vi "tdms test.vi"() -> (0 "error out":errorcluster, 3 "Pass":bool)   [LabVIEW 2015, in "tdms logger tests.lvlib"]
uses:
  tdms logger tests.lvlib
  execution/TDMS datalogger runtime.lvclass
  <vilib>/Platform/TimedLoop/XDataNode/timing_clust.ctl
  <vilib>/Platform/TimedLoop/XDataNode/nitl_modes.ctl
  <vilib>/Platform/TimedLoop/XDataNode/wakeup.ctl
  configuration/TDMS datalogger configuration.lvclass/TDMS datalogger configuration.ctl
  <vilib>/NI/Tag Bus/table/data polymorphs/write one/write Boolean.vi
  configuration/Read log directory.vi
  <vilib>/platform/TimedLoop/XDataNode/XDataNode.xnode
  configuration/TDMS datalogger configuration.lvclass
  <vilib>/NI/Tag Bus/table/data table.lvlib
  <vilib>/Platform/TimedLoop/XDataNode/XDNodeRunTimeDep.lvlib
panel:
  out "Property Names Equal?":bool
  out "Property Values Equal?":bool
  out "property values":string[][](array[string])
  out "property names":string[][](array[string])
  out "Data Equal?":bool
  out "Parsed Data":dbl[][](array[numeric])
  out "Channels Equal?":bool
  out "Groups Equal?":bool
  out "channel names":string[](array[string])
  out "group names":string[](array[string])
  out "Data Written":dbl[][](array[numeric])
  in  "iterations":i32=500
  out "max":dbl
  out "min":dbl
  in  "enable state":bool=TRUE
  out "enable found?":bool
  in  "stop":bool
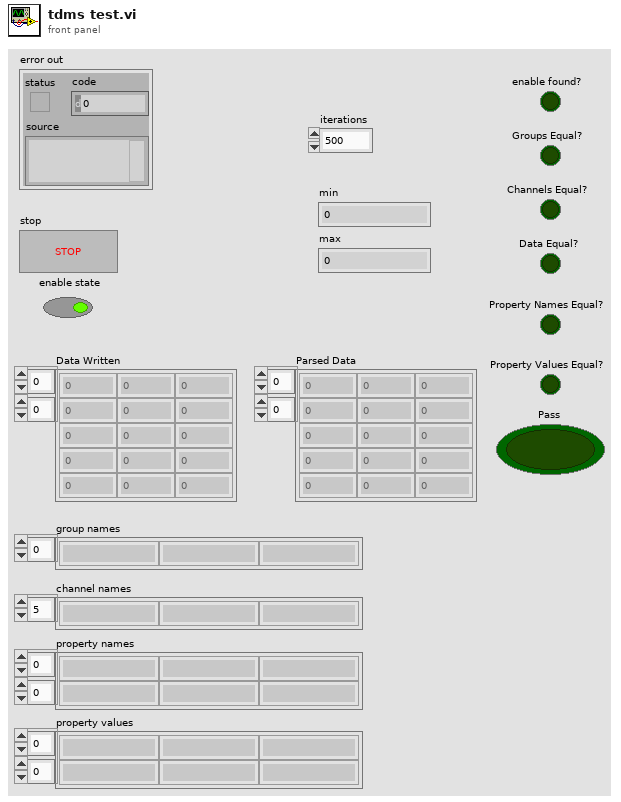
[diagram p1: front panel]
types:
  T1 = typedef "tag bus.lvlib/tag descriptor.lvclass/Data Type.ctl" = enum16{"Double", "Single", "I64", "I32", "I16", "I8", "U64", "U32", "U16", "U8", "Boolean", "String", "Array of Double", "Array of Single", "Array of I64", "Array of I32", "Array of I16", "Array of I8", "Array of U64", "Array of U32", "Array of U16", "Array of U8", "Array of Boolean", "Array of String"}
  T2 = typedef "TBM channel.lvclass/data tables.ctl" = cluster{"input data":T3, "processing parameter":T3, "processing result":T3, "output data":T3}
  T3 = typedef "tag bus.lvlib/dictionary table pair.ctl" = cluster{"data dictionary":refnum<class "data dictionary.lvclass">, "data table":T4}
  T4 = typedef "tag bus.lvlib/data table.lvlib/data table.ctl" = cluster{"Double":dbl[], "Single":sgl[], "I64":i64[], "I32":i32[], "I16":i16[], "I8":i8[], "U64":u64[], "U32":u32[], "U16":u16[], "U8":u8[], "Boolean":bool[], "String":string[], "Array of Double":cluster{"DBL Array":dbl[]}[], "Array of Single":cluster{"SGL Array":sgl[]}[], "Array of I64":cluster{"I64 Array":i64[]}[], "Array of I32":cluster{"I32 Array":i32[]}[], "Array of I16":cluster{"I16 Array":i16[]}[], "Array of I8":cluster{"I8 Array":i8[]}[], "Array of U64":cluster{"U64 Array":u64[]}[], "Array of U32":cluster{"U32 Array":u32[]}[], "Array of U16":cluster{"U16 Array":u16[]}[], "Array of U8":cluster{"U8 Array":u8[]}[], "Array of Boolean":cluster{"Boolean Array":bool[]}[], "Array of String":cluster{"String Array":string[]}[]}
  T5 = typedef "XDNodeRunTimeDep.lvlib/timing_clust.ctl" = cluster{"Expected End [f-1]":u64, "Actual End [f-1]":u64, "Finished Late? [f-1]":bool, "Expected End [i-1]":u64, "Actual End [i-1]":u64, "Finished Late? [i-1]":bool, "Expected Start [i]":u64, "Actual Start [i]":u64, "Expected Start [f]":u64, "Actual Start [f]":u64, "Source Name":string, "Structure Name":string, "Period":i64, "Deadline":i64, "Offset":i64, "Start":i64, "Priority":i32, "Timeout":i32, "Mode":T6, "Wakeup Reason":T7, "Error":errorcluster, "Source Type":string, "Secondary Source Type":string, "Global End Time":u64, "Global Start Time":u64, "Frame Duration":u64, "Iteration Duration":u64, "Assigned CPU":i32, "I/O Scan Engine Mode":u32}
  T6 = typedef "XDNodeRunTimeDep.lvlib/nitl_modes.ctl" = enum32{"No Change", "Process missed periods, maintain original phase", "Discard missed periods, maintain original phase", "Process missed periods, ignore original phase", "Discard missed periods, ignore original phase"}
  T7 = typedef "XDNodeRunTimeDep.lvlib/wakeup.ctl" = enum32{"Normal", "Aborted", "Asynchronous wakeup", "Timing source error", "Timed loop error", "Timeout"}
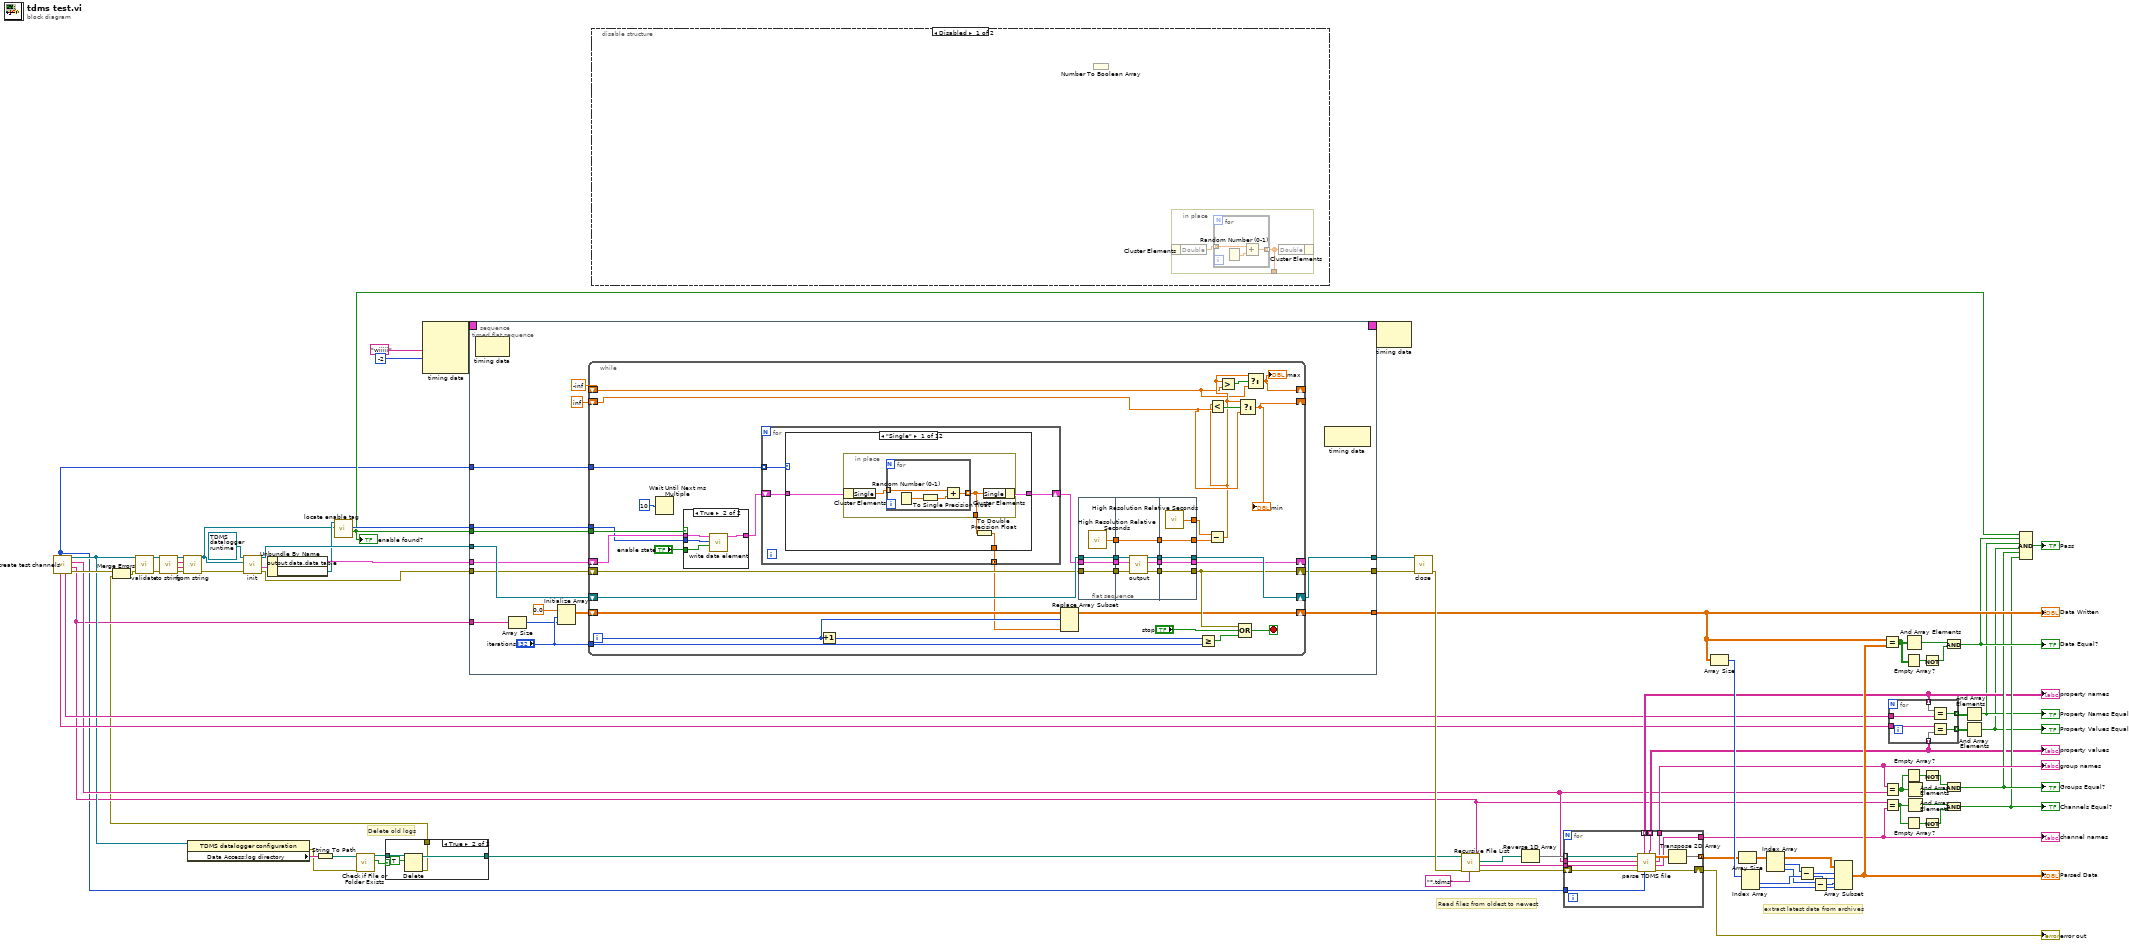
[diagram p0: block diagram]
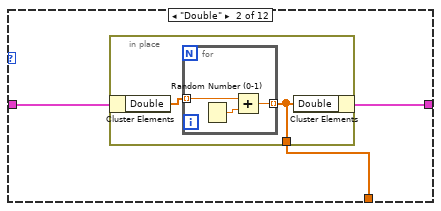
[diagram p4: hidden frame]
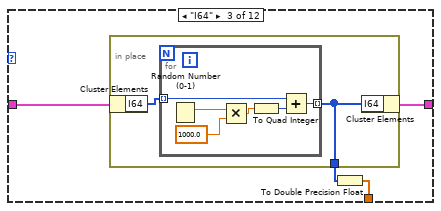
[diagram p5: hidden frame]
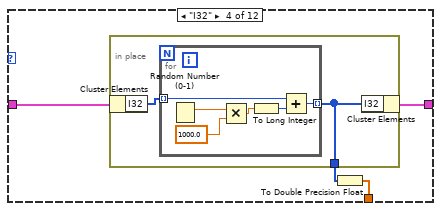
[diagram p6: hidden frame]
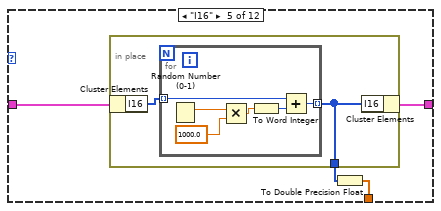
[diagram p7: hidden frame]
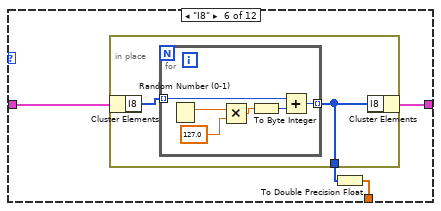
[diagram p8: hidden frame]
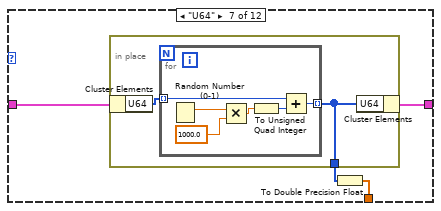
[diagram p9: hidden frame]
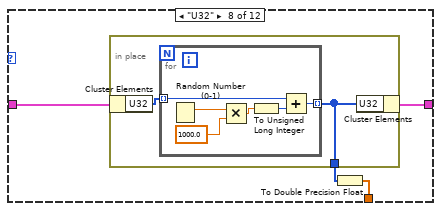
[diagram p10: hidden frame]
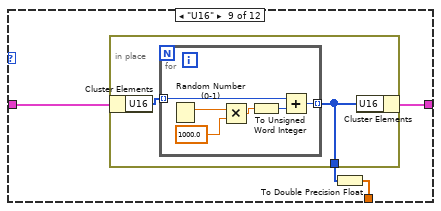
[diagram p11: hidden frame]
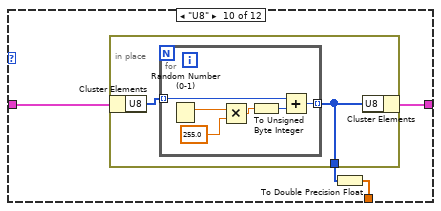
[diagram p12: hidden frame]
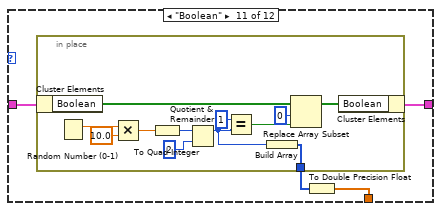
[diagram p13: hidden frame]
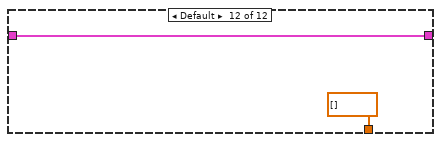
[diagram p14: hidden frame]
diagram:
  # "Delete old logs"
  # "extract latest data from archives"
  # "Read files from oldest to newest"
  n1 = call "create test channels.vi"() -> ("error out"=w15:errorcluster, "channel names"=w9:string[], "group names"=w12:string[], "TDMS datalogger configuration out"=w11:refnum<class "TDMS datalogger configuration.lvclass">, "File Property Names"=w14:string[], "File Property Values"=w13:string[], "Channel Types"=w8:T1[])  [unwired: 3 in, 2 out]
  n2 = property class="TDMS datalogger configuration"(reference=w11) -> (error out=w4:errorcluster, "Data Access:log directory"=w10:string)  [unwired: 1 in, 1 out]
  n3 = String To Path(string=w10) -> (path=w6:path)
  n4 = call <vilib>:"Check if File or Folder Exists.vi"("error in (no error)"=w4, "path"=w6) -> ("file or folder exists?"=w3:bool, "dup path"=w5:path)  [unwired: 7 in, 1 out]
  n5 = case shown="True" w3 {
    tunnel: [w79 w83] -> w7
    tunnel: [_ w81] -> w1
    tunnel: w5 -> [w79 w80]
    frame False {
    }
    frame True {
      n6 = Delete(path (use dialog)=w80, entire hierarchy (F)=TRUE) -> (deleted path=w83:path, error out=w81:errorcluster)  [unwired: 3 in, 1 out]
    }
  }
  n7 = Merge Errors(w15, w1) -> (w2:errorcluster)
  n8 = call-dynamic "validate.vi"("error in"=w2, "TDMS datalogger configuration in"=w11) -> ("error out"=w78:errorcluster, "TDMS datalogger configuration out"=w77:refnum<class "TDMS datalogger configuration.lvclass">)  [unwired: 8 in]
  n9 = call-dynamic "to string.vi"("error in"=w78, "TDMS datalogger configuration in"=w77) -> ("error out"=w75:errorcluster, "data"=w74:string, "version"=w73:string, "TDMS datalogger configuration out"=w76:refnum<class "TDMS datalogger configuration.lvclass">)  [unwired: 6 in]
  n10 = call-dynamic "from string.vi"("error in"=w75, "data"=w74, "version"=w73, "TDMS datalogger configuration in"=w76) -> ("error out"=w72:errorcluster, "TDMS datalogger configuration out"=w58:refnum<class "TDMS datalogger configuration.lvclass">)  [unwired: 6 in]
  n11 = call-dynamic "init.vi"("error in"=w72, "TBM module configuration in"=w58, "TDMS datalogger runtime in"=refnum<class "TDMS datalogger runtime.lvclass"> refnum ("TDMS datalogger runtime")) -> ("error out"=w60:errorcluster, "data allocations"=w66:T2, "TDMS datalogger runtime out"=w71:refnum<class "TDMS datalogger runtime.lvclass">)  [unwired: 5 in, 1 out]
  n12 = Unbundle By Name(w66) -> ("output data.data table"=w70:T4, "output data.data dictionary"=w65:refnum<class "data dictionary.lvclass">)
  n13 = call "locate enable tag.vi"("TDMS datalogger configuration"=w58, "data dictionary in"=w65) -> ("found?"=w37:bool, "index"=w64:i32)  [unwired: 7 in, 1 out]
  "enable found?" <- w37
  n14 = node-c288("wiiiii" ("Structure Name"), -2 ("Processor")) -> (w63:T5)  [unwired: 2 in]
  n15 = timed-sequence {
    timing: w63 -> [_]
    timing-out: [_] -> w62
    tunnel: w71 -> [w93]
    tunnel: w60 -> [w92]
    tunnel: w70 -> [w91]
    tunnel: [w90] -> w69
    tunnel: [w89] -> w68
    tunnel: w64 -> [w88]
    tunnel: w37 -> [w87]
    tunnel: [w86] -> w42
    tunnel: w9 -> [w85]
    tunnel: w8 -> [w84]
    n16 = timed-flat-sequence {
      tunnel: w93 -> [w109]
      tunnel: w92 -> [w108]
      tunnel: w91 -> [w107]
      tunnel: [w106] -> w90
      tunnel: [w105] -> w89
      tunnel: w88 -> [w104]
      tunnel: w87 -> [w103]
      tunnel: [w100] -> w86
      tunnel: w85 -> [w96]
      tunnel: w84 -> [w94]
      n17 = node-c288() -> ()  [unwired: 1 in, 1 out]
      n18 = Array Size(array=w96) -> (size(s)=w95:i32)
      n19 = Initialize Array(0.0 ("element"), "iterations", w95) -> (w99:dbl[][])
      n20 = while {
        shift-right: [w139] -> w105
        shift-left: w108 -> [w147]
        shift-right: [w146] -> w106
        shift-left: w109 -> [w148]
        shift-right: [w145] -> _
        shift-left: w107 -> [w142]
        tunnel: w104 -> [w111]
        tunnel: w103 -> [w141]
        shift-right: [w122] -> _
        shift-left: -inf -> [w124]
        shift-right: [w123] -> _
        shift-left: inf -> [w126]
        shift-right: [w120] -> w100
        shift-left: w99 -> [w119]
        tunnel: "iterations" -> [w117]
        tunnel: w94 -> [w110]
        i -> [w116]
        stop <- w140 stop-if-true
        n21 = Wait Until Next ms Multiple(millisecond multiple=u32 10) -> ()  [unwired: 1 out]
        n22 = case shown="True" w141 {
          tunnel: w142 -> [w301 w305]
          tunnel: [w301 w304] -> w112
          tunnel: w111 -> [_ w303]
          tunnel: "enable state" -> [_ w302]
          frame False {
          }
          frame True {
            n23 = call-poly <vilib>:"write data element.vi"("value"=w302, "index"=w303, "data table in"=w305) -> ("data table out"=w304:T4)  [unwired: 8 in]
          }
        }
        n24 = for {
          shift-right: [w151] -> w113
          shift-left: w112 -> [w152]
          tunnel: [w150] -> w114 mode=concatenating
          tunnel: w110 -> [w149] mode=indexing
          n25 = case shown="\"Single\"" w149 {
            tunnel: w152 -> [w155 w165 w174 w186 w198 w210 w222 w234 w246 w258 w269 w284]
            tunnel: [w156 w164 w173 w185 w197 w209 w221 w233 w245 w257 w270 w284] -> w151
            tunnel: [w153 w163 w171 w183 w195 w207 w219 w231 w243 w255 w267 dbl[] []] -> w150
            frame "Single" {
              n26 = in-place {
                in-place-border: [w157] -> w154
                n27 = in-place-cluster #1(w155) -> ("Single"=w158:sgl[])
                n28 = for {
                  tunnel: w158 -> [w162] mode=indexing
                  tunnel: [w161] -> w157 mode=indexing
                  n29 = Random Number (0-1)() -> (number: 0 to 1=w160:dbl)
                  n30 = To Single Precision Float(number=w160) -> (single precision float=w159:sgl)
                  n31 = Add(x=w162, y=w159) -> (x+y=w161:sgl)
                }
                n32 = in-place-cluster #1("Single"=w157) -> (w156:T4)
              }
              n33 = To Double Precision Float(number=w154) -> (double precision float=w153:dbl[])
            }
            frame "Double" {
              n34 = in-place {
                in-place-border: [w166] -> w163
                n35 = in-place-cluster #2(w165) -> ("Double"=w167:dbl[])
                n36 = for {
                  tunnel: w167 -> [w170] mode=indexing
                  tunnel: [w169] -> w166 mode=indexing
                  n37 = Random Number (0-1)() -> (number: 0 to 1=w168:dbl)
                  n38 = Add(x=w170, y=w168) -> (x+y=w169:dbl)
                }
                n39 = in-place-cluster #2("Double"=w166) -> (w164:T4)
              }
            }
            frame "I64" {
              n40 = in-place {
                in-place-border: [w175] -> w172
                n41 = in-place-cluster #3(w174) -> ("I64"=w176:i64[])
                n42 = for {
                  tunnel: w176 -> [w182] mode=indexing
                  tunnel: [w181] -> w175 mode=indexing
                  n43 = Random Number (0-1)() -> (number: 0 to 1=w179:dbl)
                  n44 = Multiply(x=w179, y=1000.0) -> (x*y=w178:dbl)
                  n45 = To Quad Integer(1:w178) -> (0:w180:i64)
                  n46 = Add(x=w182, y=w180) -> (x+y=w181:i64)
                }
                n47 = in-place-cluster #3("I64"=w175) -> (w173:T4)
              }
              n48 = To Double Precision Float(number=w172) -> (double precision float=w171:dbl[])
            }
            frame "I32" {
              n49 = in-place {
                in-place-border: [w187] -> w184
                n50 = in-place-cluster #4(w186) -> ("I32"=w188:i32[])
                n51 = for {
                  tunnel: w188 -> [w194] mode=indexing
                  tunnel: [w193] -> w187 mode=indexing
                  n52 = Random Number (0-1)() -> (number: 0 to 1=w191:dbl)
                  n53 = Multiply(x=w191, y=1000.0) -> (x*y=w190:dbl)
                  n54 = To Long Integer(number=w190) -> (32bit integer=w192:i32)
                  n55 = Add(x=w194, y=w192) -> (x+y=w193:i32)
                }
                n56 = in-place-cluster #4("I32"=w187) -> (w185:T4)
              }
              n57 = To Double Precision Float(number=w184) -> (double precision float=w183:dbl[])
            }
            frame "I16" {
              n58 = in-place {
                in-place-border: [w199] -> w196
                n59 = in-place-cluster #5(w198) -> ("I16"=w200:i16[])
                n60 = for {
                  tunnel: w200 -> [w206] mode=indexing
                  tunnel: [w205] -> w199 mode=indexing
                  n61 = Random Number (0-1)() -> (number: 0 to 1=w203:dbl)
                  n62 = Multiply(x=w203, y=1000.0) -> (x*y=w202:dbl)
                  n63 = To Word Integer(number=w202) -> (16bit integer=w204:i16)
                  n64 = Add(x=w206, y=w204) -> (x+y=w205:i16)
                }
                n65 = in-place-cluster #5("I16"=w199) -> (w197:T4)
              }
              n66 = To Double Precision Float(number=w196) -> (double precision float=w195:dbl[])
            }
            frame "I8" {
              n67 = in-place {
                in-place-border: [w211] -> w208
                n68 = in-place-cluster #6(w210) -> ("I8"=w212:i8[])
                n69 = for {
                  tunnel: w212 -> [w218] mode=indexing
                  tunnel: [w217] -> w211 mode=indexing
                  n70 = Random Number (0-1)() -> (number: 0 to 1=w215:dbl)
                  n71 = Multiply(x=w215, y=127.0) -> (x*y=w214:dbl)
                  n72 = To Byte Integer(number=w214) -> (8bit integer=w216:i8)
                  n73 = Add(x=w218, y=w216) -> (x+y=w217:i8)
                }
                n74 = in-place-cluster #6("I8"=w211) -> (w209:T4)
              }
              n75 = To Double Precision Float(number=w208) -> (double precision float=w207:dbl[])
            }
            frame "U64" {
              n76 = in-place {
                in-place-border: [w223] -> w220
                n77 = in-place-cluster #7(w222) -> ("U64"=w224:u64[])
                n78 = for {
                  tunnel: w224 -> [w230] mode=indexing
                  tunnel: [w229] -> w223 mode=indexing
                  n79 = Random Number (0-1)() -> (number: 0 to 1=w227:dbl)
                  n80 = Multiply(x=w227, y=1000.0) -> (x*y=w226:dbl)
                  n81 = To Unsigned Quad Integer(1:w226) -> (0:w228:u64)
                  n82 = Add(x=w230, y=w228) -> (x+y=w229:u64)
                }
                n83 = in-place-cluster #7("U64"=w223) -> (w221:T4)
              }
              n84 = To Double Precision Float(number=w220) -> (double precision float=w219:dbl[])
            }
            frame "U32" {
              n85 = in-place {
                in-place-border: [w235] -> w232
                n86 = in-place-cluster #8(w234) -> ("U32"=w236:u32[])
                n87 = for {
                  tunnel: w236 -> [w242] mode=indexing
                  tunnel: [w241] -> w235 mode=indexing
                  n88 = Random Number (0-1)() -> (number: 0 to 1=w239:dbl)
                  n89 = Multiply(x=w239, y=1000.0) -> (x*y=w238:dbl)
                  n90 = To Unsigned Long Integer(number=w238) -> (unsigned 32bit integer=w240:u32)
                  n91 = Add(x=w242, y=w240) -> (x+y=w241:u32)
                }
                n92 = in-place-cluster #8("U32"=w235) -> (w233:T4)
              }
              n93 = To Double Precision Float(number=w232) -> (double precision float=w231:dbl[])
            }
            frame "U16" {
              n94 = in-place {
                in-place-border: [w247] -> w244
                n95 = in-place-cluster #9(w246) -> ("U16"=w248:u16[])
                n96 = for {
                  tunnel: w248 -> [w254] mode=indexing
                  tunnel: [w253] -> w247 mode=indexing
                  n97 = Random Number (0-1)() -> (number: 0 to 1=w251:dbl)
                  n98 = Multiply(x=w251, y=1000.0) -> (x*y=w250:dbl)
                  n99 = To Unsigned Word Integer(number=w250) -> (unsigned 16bit integer=w252:u16)
                  n100 = Add(x=w254, y=w252) -> (x+y=w253:u16)
                }
                n101 = in-place-cluster #9("U16"=w247) -> (w245:T4)
              }
              n102 = To Double Precision Float(number=w244) -> (double precision float=w243:dbl[])
            }
            frame "U8" {
              n103 = in-place {
                in-place-border: [w259] -> w256
                n104 = in-place-cluster #10(w258) -> ("U8"=w260:u8[])
                n105 = for {
                  tunnel: w260 -> [w266] mode=indexing
                  tunnel: [w265] -> w259 mode=indexing
                  n106 = Random Number (0-1)() -> (number: 0 to 1=w263:dbl)
                  n107 = Multiply(x=w263, y=255.0) -> (x*y=w262:dbl)
                  n108 = To Unsigned Byte Integer(number=w262) -> (unsigned 8bit integer=w264:u8)
                  n109 = Add(x=w266, y=w264) -> (x+y=w265:u8)
                }
                n110 = in-place-cluster #10("U8"=w259) -> (w257:T4)
              }
              n111 = To Double Precision Float(number=w256) -> (double precision float=w255:dbl[])
            }
            frame "Boolean" {
              n112 = in-place {
                in-place-border: [w275] -> w268
                n113 = in-place-cluster #11(w269) -> ("Boolean"=w277:bool[])
                n114 = Random Number (0-1)() -> (number: 0 to 1=w282:dbl)
                n115 = Multiply(x=w282, y=10.0) -> (x*y=w280:dbl)
                n116 = To Quad Integer(1:w280) -> (0:w279:i64)
                n117 = Quotient & Remainder(x=w279, y=i64 2) -> (x-y*floor(x/y)=w273:i64)  [unwired: 1 out]
                n118 = Equal?(x=i64 1, y=w273) -> (x = y?=w271:bool)
                n119 = Build Array(w273) -> (w275:i64[])
                n120 = Replace Array Subset(array=w277, new element=w271, index=0) -> (w276:bool[])
                n121 = in-place-cluster #11("Boolean"=w276) -> (w270:T4)
              }
              n122 = To Double Precision Float(number=w268) -> (double precision float=w267:dbl[])
            }
            frame Default {
            }
          }
        }
        n123 = Increment(x=w116) -> (x+1=w118:i32)
        n124 = Replace Array Subset(array=w119, new element=w114, index (row)=w116) -> (w120:dbl[][])  [unwired: 1 in]
        n125 = flat-sequence {
          tunnel: w113 -> [w286]
          tunnel: w147 -> [w287]
          tunnel: w148 -> [w288]
          tunnel: [w288] -> w135
          tunnel: [w287] -> w134
          tunnel: [w286] -> w133
          tunnel: [w285] -> w131
          tunnel: [w293] -> w138
          tunnel: [w291] -> w137
          tunnel: [w290] -> w136
          tunnel: w135 -> [w295]
          tunnel: w134 -> [w294]
          tunnel: w133 -> [w292]
          tunnel: [w289] -> w132
          tunnel: w131 -> [w289]
          tunnel: [w298] -> w139
          tunnel: [w299] -> w145
          tunnel: [w300] -> w146
          tunnel: w138 -> [w300]
          tunnel: w137 -> [w299]
          tunnel: w136 -> [w298]
          tunnel: [w297] -> w130
          tunnel: w132 -> [w297]
          tunnel: [w296] -> w129
          frame #0 {
            n126 = call <vilib>:"High Resolution Relative Seconds.vi"() -> ("relative seconds"=w285:dbl)
          }
          frame #1 {
            n127 = call-dynamic "output.vi"("error in"=w294, "data table in"=w292, "TDMS datalogger runtime in"=w295) -> ("error out"=w290:errorcluster, "data table out"=w291:T4, "TDMS datalogger runtime out"=w293:refnum<class "TDMS datalogger runtime.lvclass">)  [unwired: 6 in]
          }
          frame #2 {
            n128 = call <vilib>:"High Resolution Relative Seconds.vi"() -> ("relative seconds"=w296:dbl)
          }
        }
        n129 = Greater Or Equal?(x=w118, y=w117) -> (x >= y?=w121:bool)
        n130 = Subtract(x=w129, y=w130) -> (x-y=w125:dbl)
        n131 = Less?(x=w125, y=w126) -> (x < y?=w127:bool)
        n132 = Greater?(x=w125, y=w124) -> (0:w128:bool)
        n133 = Compound Arithmetic op=OR(w139, "stop", w121) -> (w140:bool)
        n134 = Select(t=w125, s=w127, f=w126) -> (s? t:f=w123:dbl)
        "min" <- w123
        n135 = Select(t=w125, s=w128, f=w124) -> (s? t:f=w122:dbl)
        "max" <- w122
      }
      n136 = node-c288() -> ()  [unwired: 1 in, 1 out]
    }
  }
  "Data Written" <- w42
  n137 = disable-structure shown="Disabled" {
    frame Disabled {
      n138 = Number To Boolean Array() -> ()  [unwired: 1 in, 1 out]
      n139 = in-place {
        in-place-border: [w308] -> _
        n140 = in-place-cluster #12() -> ("Double"=w309:dbl[])  [unwired: 1 in]
        n141 = for {
          tunnel: w309 -> [w312] mode=indexing
          tunnel: [w311] -> w308 mode=indexing
          n142 = Random Number (0-1)() -> (number: 0 to 1=w310:dbl)
          n143 = Add(x=w312, y=w310) -> (x+y=w311:dbl)
        }
        n144 = in-place-cluster #12("Double"=w308) -> ()  [unwired: 1 out]
      }
    }
    frame Enabled {
    }
  }
  n145 = node-c288(w62) -> ()  [unwired: 1 out]
  n146 = call-dynamic "close.vi"("error in"=w68, "TDMS datalogger runtime in"=w69) -> ("error out"=w55:errorcluster)  [unwired: 9 in]
  n147 = call <vilib>:"Recursive File List.vi"("pattern"="*.tdms", "error in (no error)"=w55, "Folder Path"=w7) -> ("error out"=w54:errorcluster, "All Files in Dir"=w53:path[])  [unwired: 4 in, 3 out]
  n148 = Reverse 1D Array(array=w53) -> (reversed array=w52:path[])
  n149 = for {
    tunnel: w52 -> [w324] mode=indexing
    tunnel: [w318] -> w51 mode=concatenating
    tunnel: w12 -> [w322]
    tunnel: w9 -> [w321]
    shift-right: [w319] -> w40
    shift-left: w54 -> [w320]
    tunnel: [w317] -> w41
    tunnel: [w316] -> w39
    tunnel: [w315] -> w21 mode=indexing
    tunnel: [w314] -> w20 mode=indexing
    tunnel: w8 -> [w313]
    n150 = call "parse TDMS file.vi"("Channel Types"=w313, "error in"=w320, "channel name(s) in"=w321, "group names in"=w322, "file path"=w324) -> ("error out"=w319:errorcluster, "channel names"=w316:string[], "group names"=w317:string[], "Array"=w323:dbl[][], "property values"=w314:string[], "property names"=w315:string[])  [unwired: 1 in]
    n151 = Transpose 2D Array(2D array=w323) -> (transposed array=w318:dbl[][])
  }
  "error out" <- w40
  "group names" <- w41
  "channel names" <- w39
  "property names" <- w21
  "property values" <- w20
  n152 = Array Size(array=w42) -> (size(s)=w56:i32[])
  n153 = Array Size(array=w51) -> (size(s)=w50:i32[])
  n154 = Index Array(array=w56) -> (element #1=w47:i32, element #2=w46:i32)  [unwired: 2 in]
  n155 = Index Array(array=w50) -> (element #1=w48:i32, element #2=w45:i32)  [unwired: 2 in]
  n156 = Subtract(x=w48, y=w47) -> (x-y=w49:i32)
  n157 = Subtract(x=w45, y=w46) -> (x-y=w44:i32)
  n158 = Array Subset(array=w51, index (row)=w49, length (row)=w47, index (col)=w44, length (col)=w46) -> (w43:dbl[][])
  "Parsed Data" <- w43
  n159 = Equal?(x=w42, y=w43) -> (x = y?=w35:bool[][])
  n160 = Equal?(x=w41, y=w12) -> (x = y?=w23:bool[])
  n161 = Equal?(x=w9, y=w39) -> (x = y?=w22:bool[])
  n162 = for {
    tunnel: w14 -> [w330]
    tunnel: w21 -> [w329] mode=indexing
    tunnel: w20 -> [w328] mode=indexing
    tunnel: w13 -> [w327]
    tunnel: [w326] -> w18 mode=indexing
    tunnel: [w325] -> w19 mode=indexing
    n163 = Equal?(x=w329, y=w330) -> (x = y?=w325:bool[])
    n164 = Equal?(x=w327, y=w328) -> (x = y?=w326:bool[])
  }
  n165 = Empty Array?(array=w35) -> (empty?=w33:bool)
  n166 = Empty Array?(array=w23) -> (empty?=w29:bool)
  n167 = Empty Array?(array=w22) -> (empty?=w30:bool)
  n168 = And Array Elements(Boolean array=w35) -> (logical AND=w38:bool)
  n169 = And Array Elements(Boolean array=w23) -> (logical AND=w24:bool)
  n170 = And Array Elements(Boolean array=w22) -> (logical AND=w25:bool)
  n171 = Not(x=w33) -> (.not. x?=w32:bool)
  n172 = Not(x=w29) -> (.not. x?=w28:bool)
  n173 = Not(x=w30) -> (.not. x?=w31:bool)
  n174 = And(x=w38, y=w32) -> (x .and. y?=w34:bool)
  "Data Equal?" <- w34
  n175 = And(x=w28, y=w24) -> (x .and. y?=w27:bool)
  "Groups Equal?" <- w27
  n176 = And(x=w25, y=w31) -> (x .and. y?=w26:bool)
  "Channels Equal?" <- w26
  n177 = And Array Elements(Boolean array=w19) -> (logical AND=w17:bool)
  "Property Names Equal?" <- w17
  n178 = And Array Elements(Boolean array=w18) -> (logical AND=w16:bool)
  "Property Values Equal?" <- w16
  n179 = Compound Arithmetic op=AND(w37, w34, w17, w16, w27, w26) -> (→"Pass":bool)
